vi "libssh2_keepalive_config.vi"(8 "error in (no error)":errorcluster, 9 "want reply (F)":bool, 10 "interval (0 = disabled)":u32, 11 "session":T1) -> (0 "error out":errorcluster)   [LabVIEW 2017, in "libssh2.lvlib"]
doc: "Set how often keep-alive messages should be send.\n\n<B>want reply</B> indicates whether the keep-alive messages should request a response from the server.\n<B>interval</B> is the number of seconds that can pass without data being sent.\n\nNote that an interval of 1 will be treated as 2 by libssh2 to avoid some busy-loop corner-cases.\n\nThe caller is responsible for sending keep-alive messages using <B>libssh2_keepalive_send</B>."
uses:
  libssh2.lvlib
  Session Refnum.ctl
  Not A Session.vi
  <vilib>/Utility/error.llb/Error Cluster From Error Code.vi
  Global Settings.vi
  Read Session Refnum.vi
  <vilib>/Utility/semaphor.llb/Acquire Semaphore.vi
  <vilib>/Utility/semaphor.llb/Release Semaphore.vi
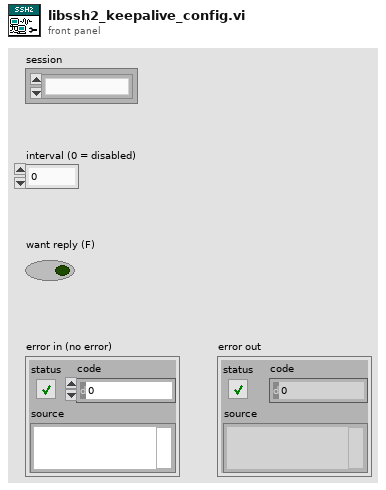
[diagram p1: front panel]
types:
  T1 = typedef "libssh2.lvlib/Session Refnum.ctl" = refnum<k1>
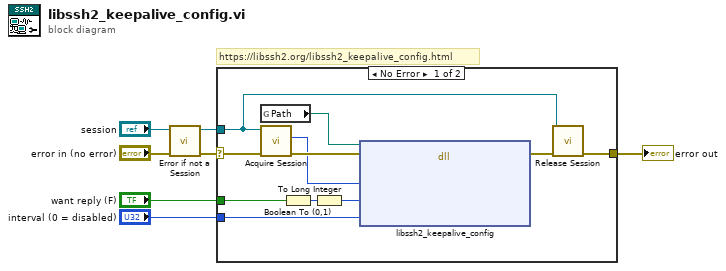
[diagram p0: block diagram]
diagram:
  # "https://libssh2.org/libssh2_keepalive_config.html"
  n1 = call "Error if not a Session.vi"("error in (no error)"="error in (no error)", "session"="session") -> ("error out"=w5:errorcluster, "session out"=w3:T1)  [unwired: 8 in]
  n2 = case shown="No Error" w5 {
    selector: w5 -> [w17 w19]
    tunnel: [w9 w19] -> w7
    tunnel: w3 -> [w8 _]
    tunnel: "interval (0 = disabled)" -> [w13 _]
    tunnel: "want reply (F)" -> [w12 _]
    frame No Error {
      n3 = global read "Global Settings.vi" "Path"() -> (w14:path)
      n4 = call "Acquire Session.vi"("error in (no error)"=w17, "session"=w8) -> ("error out"=w16:errorcluster, "LIBSSH2_SESSION*"=w15:u64)  [unwired: 7 in, 1 out]
      n5 = Boolean To (0,1)(Boolean=w12) -> (0, 1=w11:i16)
      n6 = To Long Integer(number=w11) -> (32bit integer=w10:i32)
      n7 = dll-call lib="?" fn="libssh2_keepalive_config"(path in=w14, error in=w16, "session"=w15, "want_reply"=w10, "interval"=w13) -> (error out=w18:errorcluster)  [unwired: 5 in, 1 out]
      n8 = call "Release Session.vi"("error in (no error)"=w18, "session"=w8) -> ("error out"=w9:errorcluster)  [unwired: 9 in]
    }
    frame Error {
    }
  }
  "error out" <- w7
